vi "Scheduler_Find_Ready.vi"(8 "error in (no error)":errorcluster={"status"=FALSE, "code"=0, "source"="\"\""}, 10 "active state":string, 11 "ExecutionPlan":string) -> (0 "error out":errorcluster={"status"=FALSE, "code"=0, "source"="\"\""}, 2 "status ok":bool, 3 "Ready step IDs":string)   [LabVIEW 2026]
doc: "INTENT: Select executable actions. LOGIC: Resolve ordered dependencies, joins and completed predecessors; do not start blocked branches."
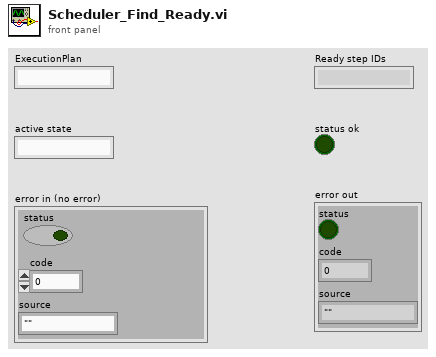
[diagram p1: front panel]
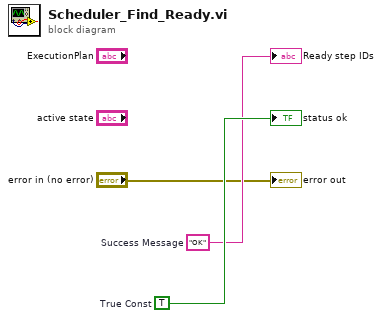
[diagram p0: block diagram]
diagram:
  w3 = TRUE  # True Const
  w2 = "OK"  # Success Message
  "Ready step IDs" <- w2
  "status ok" <- w3
  "error out" <- "error in (no error)"
